vi "PrimaryProviderExample_CreateNewWizard_Init.vi"(11 "Wizard":T1) -> (1 "Label":string, 2 "Enable Finish":bool, 3 "Enable Next":bool)   [LabVIEW 2025]
doc: "Called by the Project Explorer provider framework when an FRC Subsystem item is created."
uses:
  <resource>/Framework/Providers/API/ItemRef.ctl
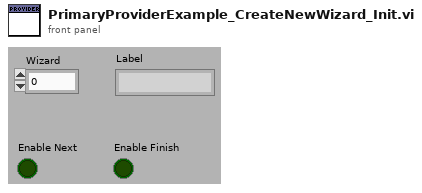
[diagram p1: front panel]
types:
  T1 = typedef "ItemRef.ctl" = u64
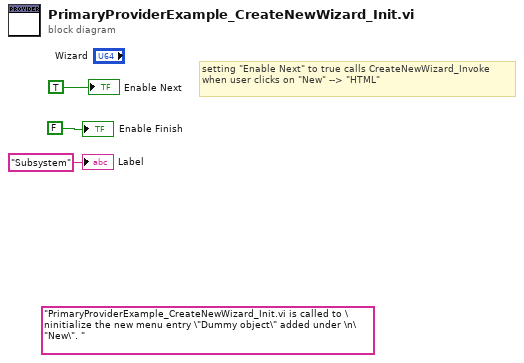
[diagram p0: block diagram]
diagram:
  (unwired) "PrimaryProviderExample_CreateNewWizard_Init.vi is called to \ninitialize the new menu entry \"Dummy object\" added under \n\"New\". " ("message")
  # "setting \"Enable Next\" to true calls CreateNewWizard_Invoke\nwhen user clicks on \"New\" --> \"HTML\""
  "Enable Next" <- TRUE
  "Enable Finish" <- FALSE
  "Label" <- "Subsystem" ("Label")
